vi "MB_WriteReg.vi"(3 "error in (no error)":errorcluster, 4 "Value":u16, 5 "Address":u16, 6 "connection ID":refnum<k5>) -> (0 "error out":errorcluster, 2 "connection ID out":refnum<k5>)   [LabVIEW 2018]
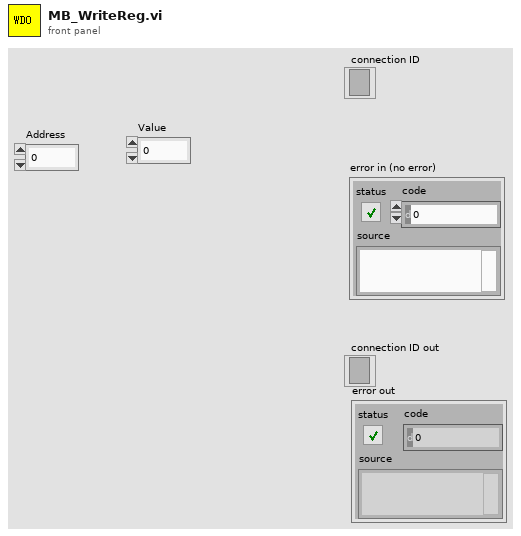
[diagram p1: front panel]
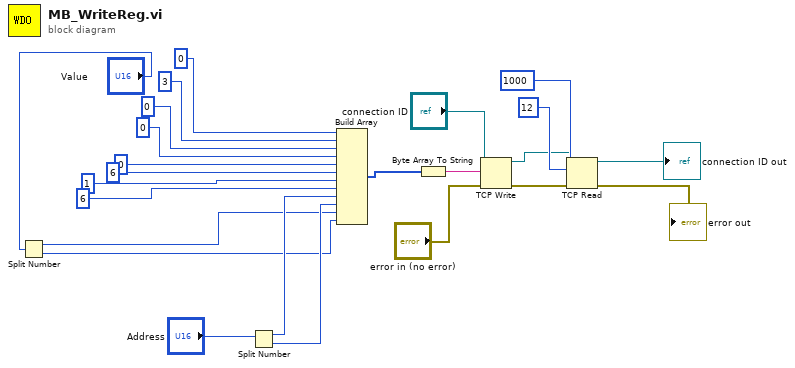
[diagram p0: block diagram]
diagram:
  n1 = Split Number(x="Value") -> (hi(x)=w2:u8, lo(x)=w1:u8)
  n2 = Split Number(x="Address") -> (hi(x)=w15:u8, lo(x)=w14:u8)
  n3 = Build Array(u8 0, u8 3, u8 0, u8 0, u8 0 ("element"), u8 6, u8 1 ("element"), u8 6, w15, w14, w2, w1) -> (w13:u8[])
  n4 = Byte Array To String(unsigned byte array=w13) -> (string=w12:string)
  n5 = TCP Write(connection ID="connection ID", data in=w12, error in (no error)="error in (no error)") -> (connection ID out=w9:refnum<k5>, error out=w8:errorcluster)  [unwired: 1 in, 1 out]
  n6 = TCP Read(connection ID=w9, bytes to read=12, error in (no error)=w8, 9:1000 ("timeout ms (25000)")) -> (connection ID out=→"connection ID out":refnum<k5>, error out=→"error out":errorcluster)  [unwired: 1 in, 1 out]
